vi "init OOB Measurement.vi"(8 "error in (no error)":errorcluster, 11 "SA Measurement in":refnum<class "SA Measurement.lvclass">) -> (0 "error out":errorcluster, 3 "SA Measurement out":refnum<class "SA Measurement.lvclass">)   [LabVIEW 2023, in "Spectrum Analyzer.lvlib" / "SA Measurement.lvclass"]
uses:
  SA Measurement.lvclass
  SA Measurement.lvclass/SA Measurement.ctl
  TYPE DEFINITION/Keysight 9020A/TYPE Measurement Preset.ctl
  Spectrum Analyzer.lvlib
  Interface_Spectrum/Interface_Spectrum.lvclass
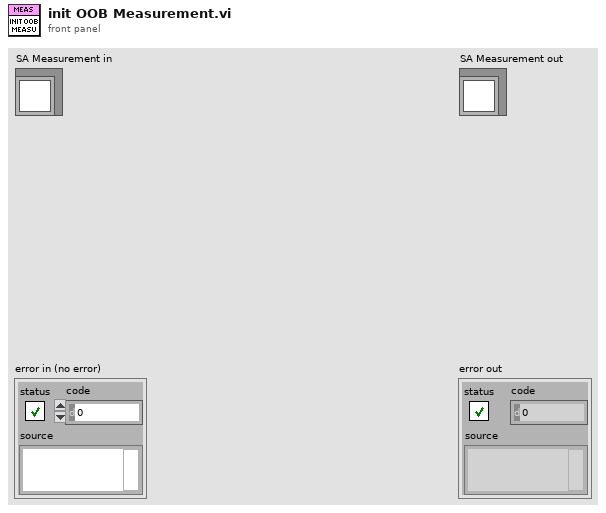
[diagram p1: front panel]
types:
  T1 = typedef "Spectrum Analyzer.lvlib/TYPE Measurement Preset.ctl" = enum16{"Sweep SA Mode", "Channel Power", "Occupied BW", "ACP", "Spurious Emission", "Spurious Emission Mask", "Burst Power (Transmit Power)"}
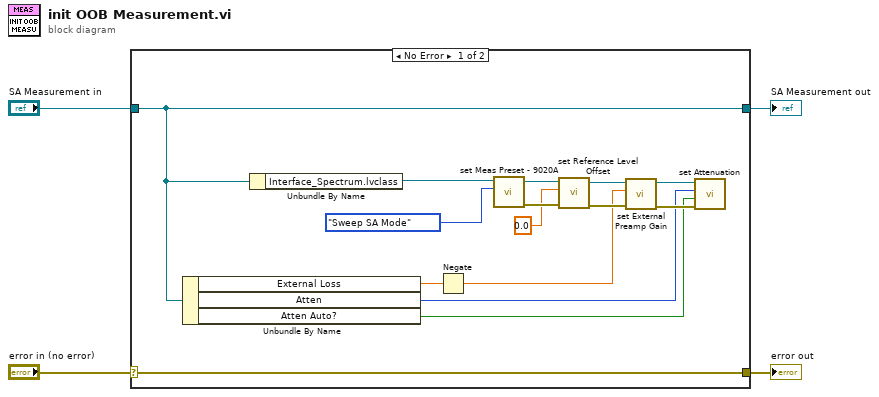
[diagram p0: block diagram]
diagram:
  n1 = case shown="No Error" "error in (no error)" {
    selector: "error in (no error)" -> [w19 w21]
    tunnel: [w19 w21] -> w3
    tunnel: [w11 w20] -> w1
    tunnel: "SA Measurement in" -> [w11 w20]
    frame No Error {
      n2 = Unbundle By Name(w11) -> ("External Loss"=w10:dbl, "Atten"=w6:i32, "Atten Auto?"=w5:bool)
      n3 = Unbundle By Name(w11) -> ("Interface_Spectrum.lvclass"=w17:refnum<class "Interface_Spectrum.lvclass">)
      n4 = Negate(x=w10) -> (-x=w9:dbl)
      n5 = call-dynamic "set Meas Preset - 9020A.vi"("Measurement Preset"=TYPE_Measurement_Preset."Sweep SA Mode", "Interface_Spectrum in"=w17) -> ("error out"=w15:errorcluster, "Interface_Spectrum out"=w16:refnum<class "Interface_Spectrum.lvclass">)  [unwired: 8 in]
      n6 = call-dynamic "set Reference Level Offset.vi"("error in (no error)"=w15, "Reference Level Offset"=0.0, "Interface_Spectrum in"=w16) -> ("error out"=w12:errorcluster, "Interface_Spectrum out"=w13:refnum<class "Interface_Spectrum.lvclass">)  [unwired: 7 in]
      n7 = call-dynamic "set External Preamp Gain.vi"("error in (no error)"=w12, "External Preamp Gain (dB)"=w9, "Interface_Spectrum in"=w13) -> ("error out"=w7:errorcluster, "Interface_Spectrum out"=w8:refnum<class "Interface_Spectrum.lvclass">)  [unwired: 7 in]
      n8 = call-dynamic "set Attenuation.vi"("error in (no error)"=w7, "Auto?"=w5, "Attenuation"=w6, "Interface_Spectrum in"=w8) -> ()  [unwired: 6 in, 2 out]
    }
    frame Error {
    }
  }
  "error out" <- w3
  "SA Measurement out" <- w1
